vi "Migrate - Read v1 Projects.vi"(8 "error in (no error)":errorcluster, 11 "Data Folder":path) -> (0 "error out":errorcluster, 1 "Default Task Names":string[](array[string]), 2 "Tasks":T1, 3 "Projects":T3)   [LabVIEW 2024]
doc: "Reads a version-1 Projects.ini: one section per project NAME with keys Task_0, Task_1 ... whose values are task name::Active or task name::Inactive. Every section except [Default] becomes a project with a new GUID, Active = TRUE and Sort Order in file order; its tasks get new GUIDs, Active from the suffix and Sort Order in key order. [Default] is not a project: its task names are returned as Default Task Names (the template for new projects).\n\nGenerated by: Claude"
uses:
  Rows/Project.ctl
  Rows/Project List.ctl
  Rows/Task.ctl
  Rows/Task List.ctl
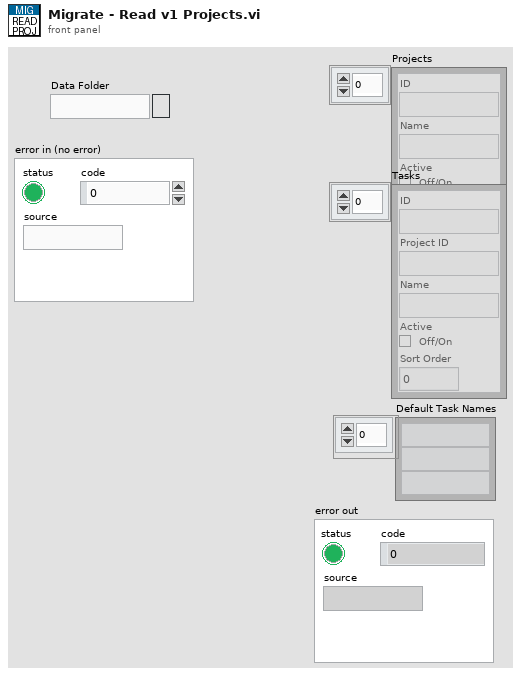
[diagram p1: front panel]
types:
  T1 = typedef "Task List.ctl" = T2[]
  T2 = typedef "Task.ctl" = cluster{"ID":string, "Project ID":string, "Name":string, "Active":bool, "Sort Order":i32}
  T3 = typedef "Project List.ctl" = T4[]
  T4 = typedef "Project.ctl" = cluster{"ID":string, "Name":string, "Active":bool, "Sort Order":i32}
  T5 = cluster{"NI GUID":string, string, "active":bool, i32}
  T6 = cluster{"NI GUID":string, "NI GUID":string, "trimmed string":string, bool, "zero":i32}
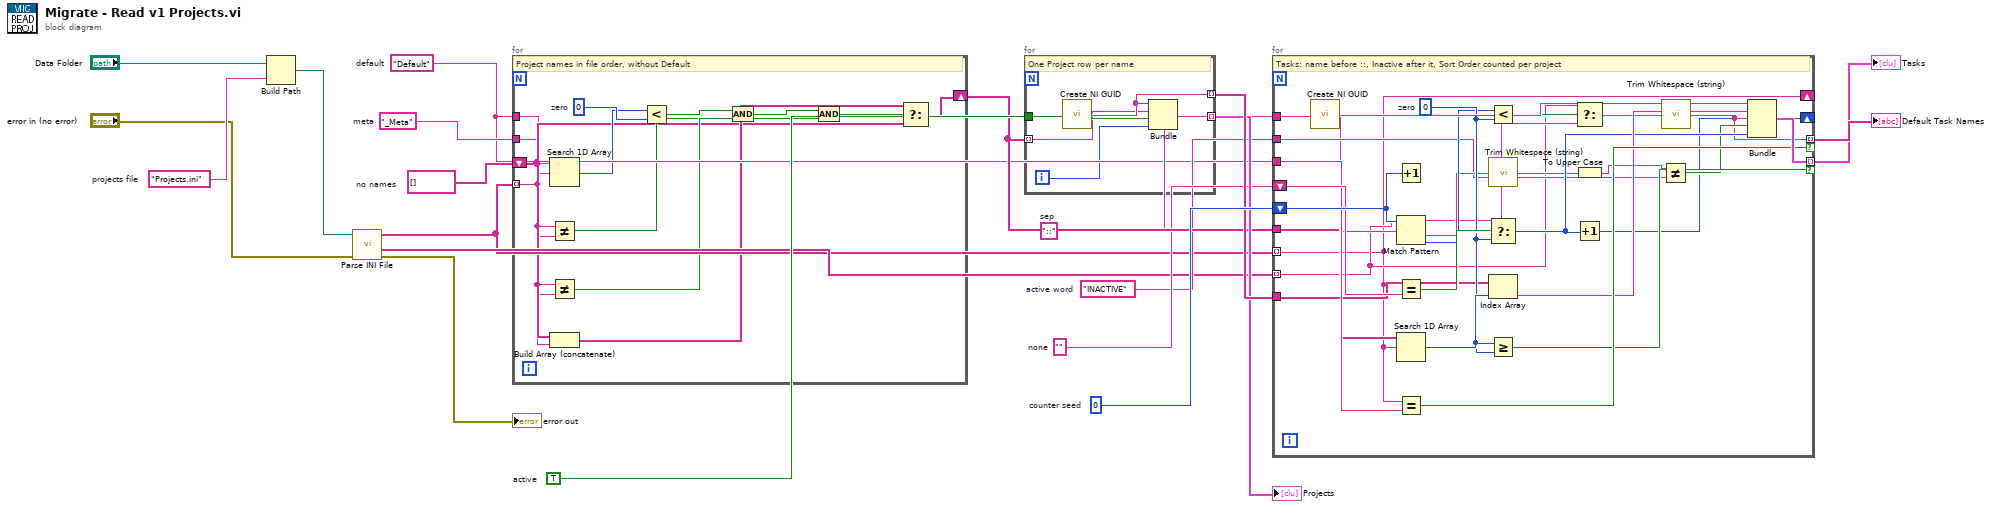
[diagram p0: block diagram]
diagram:
  w18 = 0  # counter seed
  w15 = TRUE  # active
  w13 = ""  # none
  w12 = string[] []  # no names
  w11 = "INACTIVE"  # active word
  w10 = "::"  # sep
  w9 = "_Meta"  # meta
  w8 = "Default"  # default
  w3 = "Projects.ini"  # projects file
  n1 = Build Path(base path="Data Folder", name or relative path=w3) -> (appended path=w4:path)
  n2 = call "Parse INI File.vi"("error in (no error)"="error in (no error)", "File Path"=w4) -> ("error out"=→"error out":errorcluster, "Values"=w6:string[], "Sections"=w5:string[])  [unwired: 6 in, 1 out]
  n3 = for {
    tunnel: w8 -> [w22]
    tunnel: w9 -> [w23]
    shift-right: [w25] -> w14
    shift-left: w12 -> [w24]
    tunnel: w5 -> [w21] mode=indexing
    w27 = 0  # zero
    # "Project names in file order, without Default"
    n4 = Search 1D Array(1D array=w24, element=w21) -> (index of element=w26:i32)  [unwired: 1 in]
    n5 = Not Equal?(x=w21, y=w22) -> (x != y?=w29:bool)
    n6 = Not Equal?(x=w21, y=w23) -> (x != y?=w30:bool)
    n7 = Build Array (concatenate)(w24, w21) -> (w33:string[])
    n8 = Less?(x=w26, y=w27) -> (x < y?=w28:bool)
    n9 = And(x=w28, y=w29) -> (x .and. y?=w31:bool)
    n10 = And(x=w31, y=w30) -> (x .and. y?=w32:bool)
    n11 = Select(t=w33, s=w32, f=w24) -> (s? t:f=w25:string[])
  }
  n12 = for {
    tunnel: w15 -> [w36]
    tunnel: w14 -> [w35] mode=indexing
    tunnel: [w37] -> w17 mode=indexing
    tunnel: [w38] -> w16 mode=indexing
    i -> [w34]
    # "One Project row per name"
    n13 = call <vilib>:"Create NI GUID.vi"() -> ("NI GUID"=w37:string)
    n14 = Bundle("NI GUID"=w37, w35, "active"=w36, w34) -> (w38:T5)  [unwired: 1 in]
  }
  "Projects" <- w16
  n15 = for {
    tunnel: w10 -> [w43]
    tunnel: w11 -> [w44]
    tunnel: w8 -> [w45]
    shift-right: [w39] -> _
    shift-left: w13 -> [w46]
    shift-right: [w48] -> _
    shift-left: w18 -> [w47]
    tunnel: w14 -> [w41]
    tunnel: w5 -> [w39] mode=indexing
    tunnel: w6 -> [w40] mode=indexing
    tunnel: w17 -> [w42]
    tunnel: [w55] -> w20 mode=indexing if=w64
    tunnel: [w66] -> w19 mode=indexing if=w63
    w52 = 0  # zero
    # "Tasks: name before ::, Inactive after it, Sort Order counted per project"
    n16 = call <vilib>:"Create NI GUID.vi"() -> ("NI GUID"=w65:string)
    n17 = Increment(x=w47) -> ()  [unwired: 1 out]
    n18 = Match Pattern(string=w40, regular expression=w43) -> (before substring=w49:string, after substring=w50:string, offset past match=w51:i32)  [unwired: 1 in, 1 out]
    n19 = Equal?(x=w39, y=w46) -> (x = y?=w59:bool)
    n20 = Search 1D Array(1D array=w41, element=w39) -> (index of element=w61:i32)  [unwired: 1 in]
    n21 = Equal?(x=w39, y=w45) -> (x = y?=w64:bool)
    n22 = Less?(x=w51, y=w52) -> (x < y?=w53:bool)
    n23 = call <vilib>:"Trim Whitespace (string).vi"("string"=w50) -> ("trimmed string"=w56:string)  [unwired: 1 in]
    n24 = Select(t=w47, s=w59, f=w52) -> (s? t:f=w60:i32)
    n25 = Index Array(array=w42, index=w61) -> (element=w62:string)
    n26 = Greater Or Equal?(x=w61, y=w52) -> (x >= y?=w63:bool)
    n27 = Select(t=w40, s=w53, f=w49) -> (s? t:f=w54:string)
    n28 = To Upper Case(1:w56) -> (0:w57:string)
    n29 = Increment(x=w60) -> (x+1=w48:i32)
    n30 = call <vilib>:"Trim Whitespace (string).vi"("string"=w54) -> ("trimmed string"=w55:string)  [unwired: 1 in]
    n31 = Not Equal?(x=w57, y=w44) -> (x != y?=w58:bool)
    n32 = Bundle("NI GUID"=w65, "NI GUID"=w62, "trimmed string"=w55, w58, "zero"=w60) -> (w66:T6)  [unwired: 1 in]
  }
  "Tasks" <- w19
  "Default Task Names" <- w20
